vi "Initialization.vi"(8 "error in (no error)":errorcluster, 9 "UI Refs":T1, 10 "user event":T2, 11 "PG":refnum<class "Pressure Gain.lvclass">) -> (0 "error out":errorcluster, 3 "PG out":refnum<class "Pressure Gain.lvclass">)   [LabVIEW 2025, in "Flow Grind.lvlib" / "Pressure Gain.lvclass"]
uses:
  Pressure Gain.lvclass
  Users/Public/Documents/Sandia National Labs/TSS Plugin/CEF.lvlibp/Node/UserEventRef.ctl
  Users/Public/Documents/Sandia National Labs/TSS Plugin/Tests/XY Plotter.lvlibp/XY  Plotter/XY Plotter.lvclass
  Users/Public/Documents/Sandia National Labs/TSS Plugin/CEF.lvlibp/Node/CEF_Node.lvclass
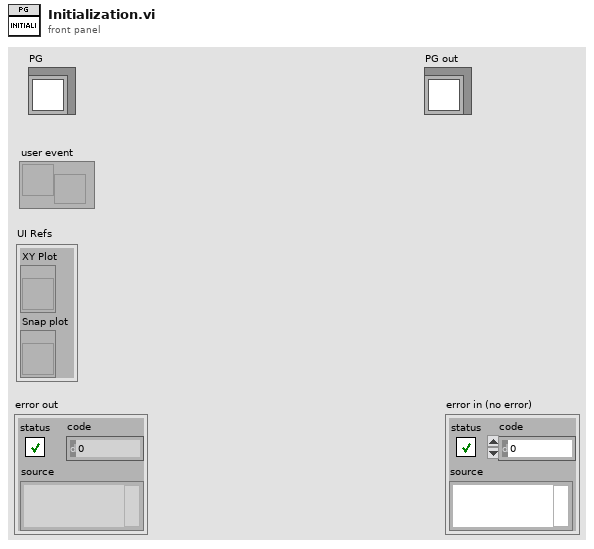
[diagram p1: front panel]
types:
  T1 = cluster{"XY Plot":refnum<vi>, "Snap plot":refnum<vi>}
  T2 = typedef "CEF.lvlibp/CEF_Node.lvclass/UserEventRef.ctl" = refnum<user-event>
  T3 = cluster{"Name":string, "Color":u32, "Style":u8, "Point Style":u8, "Name Visible":bool, "Allow Drag":bool, "Annotation Mode":u32, "Plot":i32, "Index":i32, "Position":cluster{"X":dbl, "Y":dbl}, "X Scale":u32, "Y Scale":u32, "Show Arrow":bool, "Lock Name":bool, "Plot Area":i32, "Label Offset":cluster{"X":dbl, "Y":dbl}}
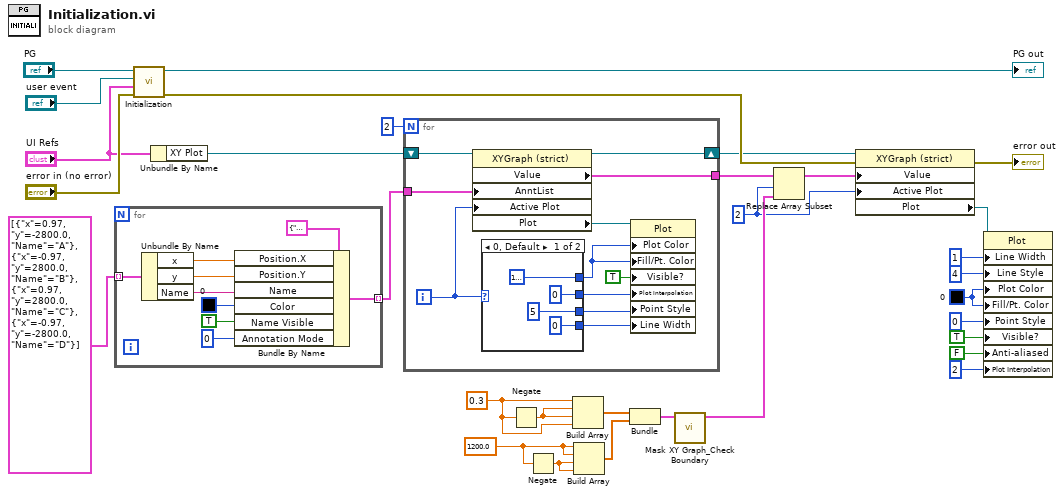
[diagram p0: block diagram]
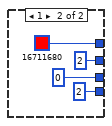
[diagram p2: hidden frame]
diagram:
  w7 = 2 ("index")
  w9 = u32 0 ("Plot Color")
  w18 = 1200.0 ("y")
  w19 = 0.3 ("x")
  n1 = for {
    tunnel: cluster{"x":dbl, "y":dbl, "Name":string}[] [{"x"=0.97, "y"=-2800.0, "Name"="A"}, {"x"=-0.97, "y"=2800.0, "Name"="B"}, {"x"=0.97, "y"=2800.0, "Name"="C"}, {"x"=-0.97, "y"=-2800.0, "Name"="D"}] -> [w35] mode=indexing
    tunnel: [w36] -> w5 mode=indexing
    n2 = Unbundle By Name(w35) -> ("x"=w33:dbl, "y"=w32:dbl, "Name"=w34:string)
    n3 = Bundle By Name(cluster=T3 {"Name"="", "Color"=0, "Style"=0, "Point Style"=0, "Name Visible"=FALSE, "Allow Drag"=FALSE, "Annotation Mode"=0, "Plot"=0, "Index"=0, "Position"={"X"=0.0, "Y"=0.0}, "X Scale"=0, "Y Scale"=0, "Show Arrow"=FALSE, "Lock Name"=FALSE, "Plot Area"=0, "Label Offset"={"X"=0.0, "Y"=0.0}}, "Position.X"=w33, "Position.Y"=w32, "Name"=w34, "Color"=u32 0, "Name Visible"=TRUE, "Annotation Mode"=u32 0) -> (w36:T3)
  }
  n4 = call-parent "Initialization.vi"("error in"="error in (no error)", "UI Refs"="UI Refs", "user event"="user event", "XY Plotter"="PG") -> ("error out"=w3:errorcluster, "XY Plotter out"=→"PG out":refnum<class "Pressure Gain.lvclass">)  [unwired: 6 in]
  n5 = Unbundle By Name("UI Refs") -> ("XY Plot"=w6:refnum<vi>)
  n6 = for {
    N: 2 -> [_]
    tunnel: w5 -> [w42]
    shift-right: [w44] -> w2
    shift-left: w6 -> [w51]
    tunnel: [w41] -> w1
    i -> [w49]
    n7 = property class="XYGraph (strict)"(reference=w51, "AnntList"=w42, "Active Plot"=w49) -> (reference out=w44:refnum<vi>, "Value"=w41:cluster{"Wavenumber":dbl[], "Data":dbl[]}[], "Plot"=w43:refnum<vi>)  [unwired: 1 in, 1 out]
    n8 = case shown="0, Default" w49 {
      tunnel: [u32 16777224 ("Plot.Plot Color") u32 16711680 ("Plot.Plot Color")] -> w48
      tunnel: [u8 0 ("Plot Interpolation") u8 2 ("Plot Interpolation")] -> w47
      tunnel: [u8 5 ("Point Style") u8 0 ("Point Style")] -> w46
      tunnel: [u8 0 ("Line Width") u8 2 ("Line Width")] -> w45
      frame 0, Default {
      }
      frame 1 {
      }
    }
    n9 = property class="Plot"(reference=w43, "Plot Color"=w48, "Fill/Pt. Color"=w48, "Visible?"=TRUE ("Visible"), "Plot Interpolation"=w47, "Point Style"=w46, "Line Width"=w45) -> ()  [unwired: 1 in, 2 out]
  }
  n10 = Negate(x=w19) -> (-x=w20:dbl)
  n11 = Negate(x=w18) -> (-x=w17:dbl)
  n12 = Build Array(w19, w20, w20, w19) -> (w25:dbl[])
  n13 = Build Array(w18, w18, w17, w17) -> (w24:dbl[])
  n14 = Bundle(w25, w24) -> (w23:cluster{dbl[], dbl[]})  [unwired: 1 in]
  n15 = call "Mask XY Graph_Check Boundary.vi"("Boundary"=w23) -> ("Closed Boundary"=w22:cluster{"X":dbl[], "Y":dbl[]})  [unwired: 9 in, 1 out]
  n16 = Replace Array Subset(array=w1, new element=w22, index=w7) -> (w16:cluster{"Wavenumber":dbl[], "Data":dbl[]}[])
  n17 = property class="XYGraph (strict)"(reference=w2, error in=w3, "Value"=w16, "Active Plot"=w7) -> (error out=→"error out":errorcluster, "Plot"=w8:refnum<vi>)  [unwired: 1 out]
  n18 = property class="Plot"(reference=w8, "Line Width"=u8 1, "Line Style"=u8 4, "Plot Color"=w9, "Fill/Pt. Color"=w9, "Point Style"=u8 0, "Visible?"=TRUE ("Visible"), "Anti-aliased"=FALSE, "Plot Interpolation"=u8 2) -> ()  [unwired: 1 in, 2 out]
